vi "Set Columns.vi"() -> ()   [LabVIEW 2020]
doc: "Development tool: sizes a multicolumn listbox by its columns and rows, which LabVIEW does not let Bounds do (a multicolumn listbox has no writable size). Sets the width of each column (Widths, one per column) and then the number of visible columns (as many as Widths) and the number of visible rows, then saves the VI. The listbox is then as wide as its columns plus its frame (and its vertical scroll bar). A VI that writes Number of Columns at run time keeps these widths. Run it on a VI that is not running."
panel:
  out "error out":errorcluster
  out "size":i32[](array[numeric])
  in  "Rows":i32=10
  in  "Widths":i32[](array[numeric])
  in  "Label":string
  in  "VI":path
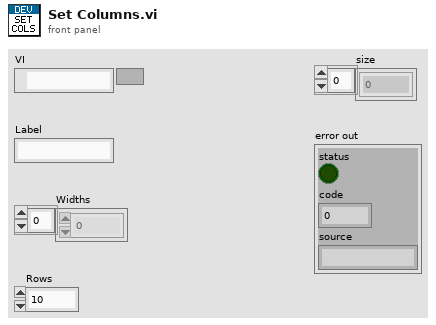
[diagram p1: front panel]
types:
  T1 = typedef "LVBoundsTypeDef.ctl" = cluster{"Width":u32, "Height":u32}
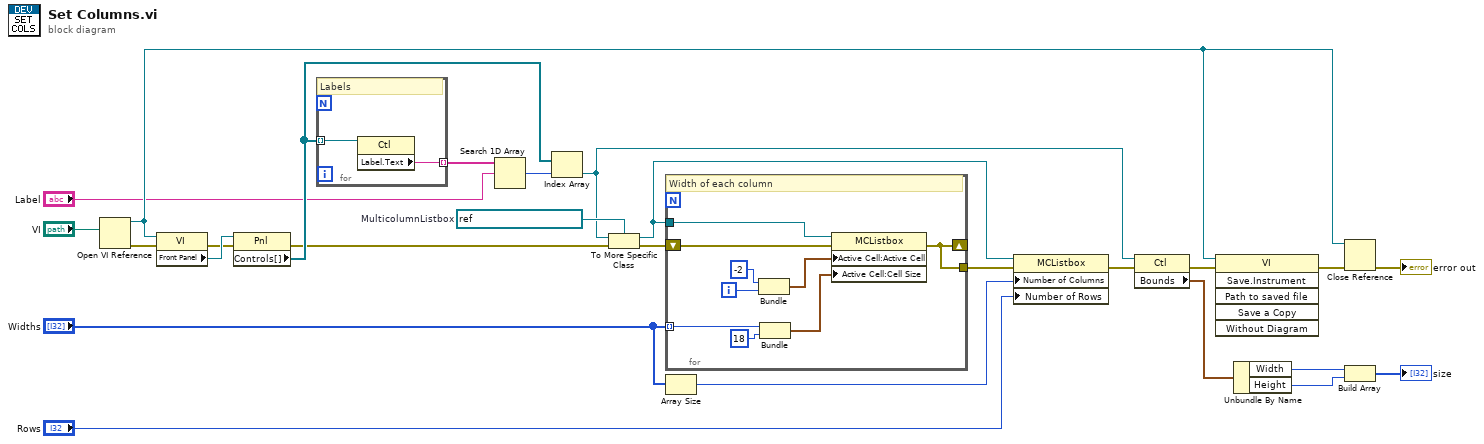
[diagram p0: block diagram]
diagram:
  w14 = refnum<vi> refnum  # MulticolumnListbox
  n1 = Open VI Reference(vi path="VI") -> (vi reference=w5:refnum<vi>, error out=w6:errorcluster)  [unwired: 5 in]
  n2 = property class="VI"(reference=w5, error in=w6) -> (error out=w7:errorcluster, "Front Panel"=w8:refnum<vi>)  [unwired: 1 out]
  n3 = property class="Pnl"(reference=w8, error in=w7) -> (error out=w9:errorcluster, "Controls[]"=w10:refnum<vi>[])  [unwired: 1 out]
  n4 = for {
    tunnel: w10 -> [w27] mode=indexing
    tunnel: [w28] -> w11 mode=indexing
    # "Labels"
    n5 = property class="Ctl"(reference=w27) -> ("Label.Text"=w28:string)  [unwired: 1 in, 2 out]
  }
  n6 = Search 1D Array(1D array=w11, element="Label") -> (index of element=w12:i32)  [unwired: 1 in]
  n7 = Index Array(array=w10, index=w12) -> (element=w13:refnum<vi>)
  n8 = To More Specific Class(target class=w14, reference=w13, error in=w9) -> (specific class reference=w15:refnum<vi>, error out=w16:errorcluster)
  n9 = for {
    tunnel: "Widths" -> [w30] mode=indexing
    tunnel: w15 -> [w31]
    shift-right: [w33] -> _
    shift-left: w16 -> [w32]
    tunnel: [w33] -> w19
    i -> [w29]
    # "Width of each column"
    n10 = Bundle(-2, w29) -> (w36:cluster{i32, i32})  [unwired: 1 in]
    n11 = Bundle(w30, 18) -> (w37:cluster{i32, i32})  [unwired: 1 in]
    n12 = property class="MCListbox"(reference=w31, error in=w32, "Active Cell:Active Cell"=w36, "Active Cell:Cell Size"=w37) -> (error out=w33:errorcluster)  [unwired: 1 out]
  }
  n13 = Array Size(array="Widths") -> (size(s)=w17:i32)
  n14 = property class="MCListbox"(reference=w15, error in=w19, "Number of Columns"=w17, "Number of Rows"="Rows") -> (error out=w18:errorcluster)  [unwired: 1 out]
  n15 = property class="Ctl"(reference=w13, error in=w18) -> (error out=w20:errorcluster, "Bounds"=w21:T1)  [unwired: 1 out]
  n16 = invoke class="VI" method="Save.Instrument"(reference=w5, error in=w20) -> (error out=w25:errorcluster)  [unwired: 4 in, 5 out]
  n17 = Unbundle By Name(w21) -> ("Width"=w22:u32, "Height"=w23:u32)
  n18 = Close Reference(reference=w5, error in (no error)=w25) -> (error out=→"error out":errorcluster)
  n19 = Build Array(w22, w23) -> (→"size":u32[])
